vi "Benchmark mupExpr_eval.vi"(8 "error in (no error)":errorcluster, 10 "Iterations":i32=100000, 11 "Expression":string="5*x^2+2*x+20") -> (0 "error out":errorcluster, 2 "x":dbl[](array[numeric]), 3 "y":dbl[](array[numeric]), 5 "dt average":dbl)   [LabVIEW 2015]
uses:
  mupExpr/mupExpr.lvclass
  mupExpr/mupExpr.lvclass/mupExpr.ctl
  mupLib/mupEval.vi
  mupLib/mupSetVarValue.vi
  mupLib/mupCheckError.vi
  <vilib>/Utility/error.llb/Error Cluster From Error Code.vi
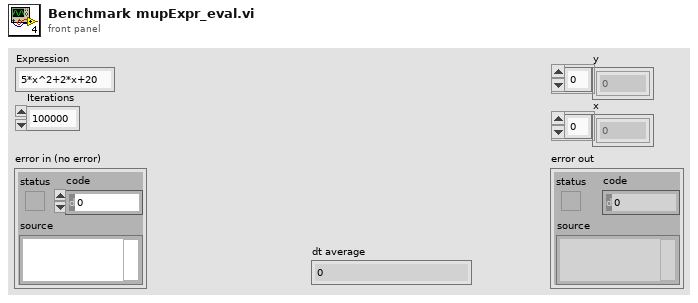
[diagram p1: front panel]
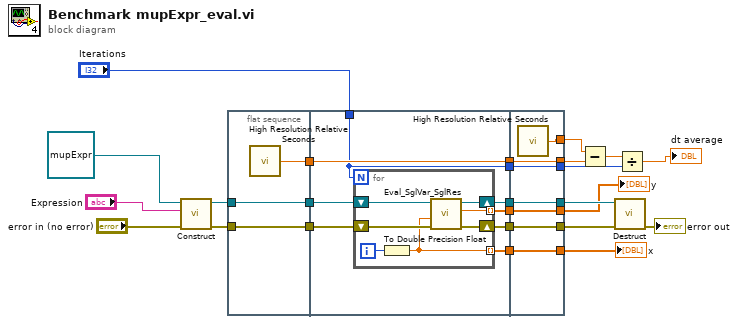
[diagram p0: block diagram]
diagram:
  n1 = call-dynamic "Construct.vi"("error in (no error)"="error in (no error)", "Expression"="Expression", "muExpr in"=refnum<class "mupExpr.lvclass"> refnum) -> ("error out"=w23:errorcluster, "mupExpr out"=w24:refnum<class "mupExpr.lvclass">)  [unwired: 5 in, 2 out]
  n2 = flat-sequence {
    tunnel: w23 -> [w27]
    tunnel: w24 -> [w28]
    tunnel: [w28] -> w16
    tunnel: [w27] -> w15
    tunnel: [w26] -> w9
    tunnel: w16 -> [w36]
    tunnel: w15 -> [w35]
    tunnel: [w34] -> w14
    tunnel: [w33] -> w13
    tunnel: [w32] -> w12
    tunnel: [w31] -> w11
    tunnel: [w30] -> w10
    tunnel: w9 -> [w30]
    tunnel: "Iterations" -> [w29]
    tunnel: [w29] -> w3
    tunnel: [w47] -> w19
    tunnel: [w48] -> w20
    tunnel: [w49] -> w21
    tunnel: [w50] -> w22
    tunnel: w14 -> [w50]
    tunnel: w13 -> [w49]
    tunnel: w12 -> [w48]
    tunnel: w11 -> [w47]
    tunnel: [w46] -> w7
    tunnel: w10 -> [w46]
    tunnel: [w45] -> w8
    tunnel: [w44] -> w4
    tunnel: w3 -> [w44]
    frame #0 {
      n3 = call <vilib>:"High Resolution Relative Seconds.vi"() -> ("relative seconds"=w26:dbl)
    }
    frame #1 {
      n4 = for {
        N: w29 -> [_]
        shift-right: [w41] -> w33
        shift-left: w35 -> [w42]
        shift-right: [w40] -> w34
        shift-left: w36 -> [w39]
        tunnel: [w38] -> w32 mode=indexing
        tunnel: [w37] -> w31 mode=indexing
        i -> [w43]
        n5 = To Double Precision Float(number=w43) -> (double precision float=w37:dbl)
        n6 = call "Eval_SglVar_SglRes.vi"("error in (no error)"=w42, "varValue"=w37, "muExpr in"=w39) -> ("error out"=w41:errorcluster, "Result"=w38:dbl, "muExpr out"=w40:refnum<class "mupExpr.lvclass">)  [unwired: 6 in]
      }
    }
    frame #2 {
      n7 = call <vilib>:"High Resolution Relative Seconds.vi"() -> ("relative seconds"=w45:dbl)
    }
  }
  n8 = Subtract(x=w8, y=w7) -> (x-y=w5:dbl)
  n9 = call-dynamic "Destruct.vi"("error in (no error)"=w21, "muExpr in"=w22) -> ("error out"=→"error out":errorcluster)  [unwired: 9 in]
  n10 = Divide(x=w5, y=w4) -> (x/y=→"dt average":dbl)
  "y" <- w20
  "x" <- w19
